vi "pwmSetClock.vi"(8 "error in (no error)":errorcluster, 11 "Divisor":i32) -> (0 "error out":errorcluster)   [LabVIEW 2020, in "wiringPi.lvlib"]
doc: "<b>_______________________________________________________________</b>\n** Author: Juan José Villacorta\n** LabVIEW wrapper for C library <b> wiringPi </b>,\n** https://github.com/WiringPi/WiringPi\n<b>_______________________________________________________________</b>\n\n/*\n * pwmWrite:\n * Changes the PWM value of the pin. Possible values are 0 -> { PWM Range }\n *********************************************************************************\n */"
uses:
  wiringPi.lvlib
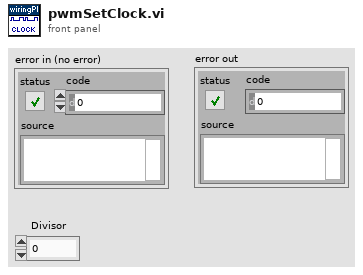
[diagram p1: front panel]
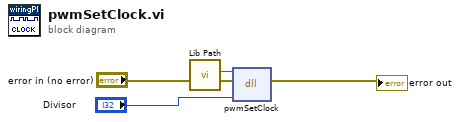
[diagram p0: block diagram]
diagram:
  n1 = call "Lib Path.vi"() -> ("path out"=w1:path)  [unwired: 11 in]
  n2 = dll-call lib="libLVwiringPI.so" fn="pwmSetClock"(path in=w1, error in="error in (no error)", "mode"="Divisor") -> (error out=→"error out":errorcluster)  [unwired: 3 in, 1 out]
